vi "Start Condition - Saturation Time (SubVI) (1).vi"(6 "Enum":T1(ring), 8 "error in (no error)":errorcluster, 9 "Time":dbl, 10 "Select":i32, 11 "Cluster in":T2 {"M Event" items=["Stop", "Running", "PID", "Up Limit", "Down Limit", "Load Limit"]; "Test Type" items=["Please Select", "Triaxial Shear", "Triaxial UU", "Shearbox", "Permeability", "Consolidation (Stepped Loading)/Swelling", "Saturation (Incremental)", "User Defined", "UCT", "Isotropic Consolidation", "Swelling Pressure", "B-Check", "Saturation (Step Increment)", "Saturation (Ramp)"]; "Data"."Test Type" items=["Please Select", "Triaxial Shear", "Triaxial UU", "Shearbox", "Permeability", "Consolidation (Stepped Loading)/Swelling", "Saturation (Incremental)", "User Defined", "UCT", "Isotropic Consolidation", "Swelling Pressure", "B-Check", "Saturation (Step Increment)", "Saturation (Ramp)"]}) -> (0 "error out":errorcluster, 3 "Cluster out":T2 {"M Event" items=["Stop", "Running", "PID", "Up Limit", "Down Limit", "Load Limit"]; "Test Type" items=["Please Select", "Triaxial Shear", "Triaxial UU", "Shearbox", "Permeability", "Consolidation (Stepped Loading)/Swelling", "Saturation (Incremental)", "User Defined", "UCT", "Isotropic Consolidation", "Swelling Pressure", "B-Check", "Saturation (Step Increment)", "Saturation (Ramp)"]; "Data"."Test Type" items=["Please Select", "Triaxial Shear", "Triaxial UU", "Shearbox", "Permeability", "Consolidation (Stepped Loading)/Swelling", "Saturation (Incremental)", "User Defined", "UCT", "Isotropic Consolidation", "Swelling Pressure", "B-Check", "Saturation (Step Increment)", "Saturation (Ramp)"]})   [LabVIEW 2019]
uses:
  Controls/RunTest - Data Structure.ctl
  Controls/Test Panel - Data Structure.ctl
  Controls/Station - Test Type.ctl
  <vilib>/Utility/miscctls.llb/LVRowAndColumnTypeDef.ctl
  Controls/RunTest - Calculate Data.ctl
  <vilib>/httpClient/ClientHandle.ctl
  Controls/RunTest - Start Condition.ctl
  Controls/RunTest - Stop Condition.ctl
  Controls/UDP - Event.ctl
  <vilib>/httpClient/LabVIEWHTTPClient.lvlib
types:
  T1 = enum16{"Saturation", "B-Check", "Sat Step", "Sat Ramp"}
  T2 = typedef "RunTest - Data Structure.ctl" = cluster{"Test Plan":string[], "PlanRow":i32, "Device Name":string[], "Timeout":i32, "Start?":bool, "Pause?":bool, "IP Address":string[], "LogRow":i32, "Logtype":u16, "Log Elapse":sgl, "Data":T3, "Stop log?":bool, "tdms":refnum<k34>, "Sensor Data":sgl[], "Start time":timestamp, "Prev Log Elapse":u32, "Plot":u16, "X-Axis":u16[], "Y-Axis":u16[], "XY":cluster{"X":dbl, "Y":dbl}[][], "End Stage?":bool, "1run":bool, "Condition":u16[], "Start Con":bool, "Log Con":bool, "Stop Con":bool, "Start Elapse":dbl, "Start Load":dbl, "Motor":i32, "StartRow":i32, "number log":i32, "Dir":bool, "Start time test":timestamp, "Auto":bool, "Check return?":bool, "Inv":cluster{"M":i32[], "Bool":bool[]}, "tdms temp":refnum<k34>, "Zero?":bool, "Plot Timer":dbl, "1st Run":bool, "TDMS Path":path, "MaxLoad":dbl, "Log Timer":sgl[], "Test Type":T4, "Log Sensor":string[], "Save?":bool, "1st Log":bool, "Y-Axis 2":u16[], "On Y-Axis 2":bool, "Decimal":u8[], "Init":cluster{"PWP TS":sgl, "Load TS":sgl, "Volume TS":sgl, "Disp TS":sgl, "CP":sgl, "Vol In":sgl, "Vol Out":sgl, "Load UCT":sgl, "Disp UCT":sgl, "PWP Sat":sgl, "CP Sat":sgl, "Volume IsoCons":sgl, "PWP IsoCons":sgl, "PWP TUU":sgl, "Load TUU":sgl, "Volume TUU":sgl, "Disp TUU":sgl, "Load Cons":sgl, "Disp Cons":sgl, "Volume Sat":sgl, "Vertical Load SB":sgl, "Vertical Disp SB":sgl, "H Disp SB":sgl, "H Load SB":sgl, "PWP BC":sgl, "CP BC":sgl, "PWP Sat Step":sgl, "CP Sat Step":sgl, "Volume Sat Step":sgl, "PWP Sat Ramp":sgl, "CP Sat Ramp":sgl, "Volume Sat Ramp":sgl}, "Calc":T6, "Device Index":i32[], "Channel Index":i32[], "http ref":T7, "fileid":string, "Step Cons":cluster{"V Stress":sgl, "H Settlement":sgl}, "RunTest":bool, "Graph Last":i32, "Init?":bool, "Datalog":bool[], "Start":T8, "Stop":T9, "Running?":bool, "StartTime":dbl, "Log Prev Time":dbl, "KeyName":string[], "Test RunTime":dbl, "Log Prev Axial":dbl, "M Event":T10[], "Last Log":bool, "popup":bool, "PreStart UU":bool, "PreStart Sat":bool, "PreStart BC":bool, "PreStart Sat Step":bool, "PreStart Sat Ramp":bool, "Prev Sat IP":string}
  T3 = typedef "Test Panel - Data Structure.ctl" = cluster{"Station":string, "Sample ID":string, "Job No":string, "Job Description":string, "Filename":string, "Test Type":T4, "Speciment No":string, "Depth":string, "Height":string, "Diameter/Length":string, "Weight":string, "Test Parameter":string, "Station[]":string[], "Edit Pos":T5, "Edit Pos Prev":T5, "Area":string, "Path":string, "sample_id":string}
  T4 = typedef "Station - Test Type.ctl" = u16
  T5 = typedef "LVRowAndColumnTypeDef.ctl" = cluster{"Row":i32, "Column":i32}
  T6 = typedef "RunTest - Calculate Data.ctl" = cluster{"TS":cluster{"Change PWP":sgl, "Change Vol":sgl, "Axial Load":sgl, "CiL":sgl, "Deviator":sgl, "Axial Strain":sgl, "MaxDeviator":sgl, "SS":sgl, "CAS":sgl}, "TUU":cluster{"Change PWP":sgl, "Axial Load":sgl, "CiL":sgl, "Deviator":sgl, "Axial Strain":sgl, "MaxDeviator":sgl}, "Sat":cluster{"B Value":sgl, "PWP Diss":sgl, "CPP":sgl, "CV":sgl}, "Per":cluster{"Change Vol In":sgl, "Change Vol Out":sgl, "Mean Vol":sgl, "Gradient Pressure":sgl, "Outlet Flow":sgl, "Inlet Flow":sgl, "I X1":sgl, "I X2":sgl, "I Y1":sgl, "I Y2":sgl, "O X1":sgl, "O X2":sgl, "O Y1":sgl, "O Y2":sgl}, "Step Cons":cluster{"V Stress":sgl, "H Settlement":sgl, "Total H Settle":sgl, "Prev Total H":sgl}, "UCT":cluster{"ALC":sgl, "H Change":sgl, "Deviator":sgl, "Axial Strain":sgl, "V Stress":sgl, "MaxDeviator":sgl}, "ISO Cons":cluster{"CPP":sgl, "PWP Diss":sgl, "CV":sgl, "VS":sgl}, "SB":cluster{"Speci LenC":sgl, "Shear Strain":sgl, "H LC":sgl, "Normal Stress":sgl, "Shear Stress":sgl, "MaxShear":sgl}, "BC":cluster{"B Value":sgl, "PWP Diss":sgl, "CPP":sgl, "CV":sgl}, "Sat Step":cluster{"B Value":sgl, "PWP Diss":sgl, "CPP":sgl, "CV":sgl}, "Sat Ramp":cluster{"B Value":sgl, "PWP Diss":sgl, "CPP":sgl, "CV":sgl}, "Prev Log":string[]}
  T7 = typedef "LabVIEWHTTPClient.lvlib/ClientHandle.ctl" = refnum<k1>
  T8 = typedef "RunTest - Start Condition.ctl" = cluster{"Cons":cluster{"VS":dbl, "Delay":bool, "No Delay":dbl}, "Sat":cluster{"CP":dbl, "BP":dbl, "StartBP":bool, "Target CP":bool, "Target BP":bool}, "Iso":cluster{"Select":dbl, "BP":dbl, "IC2":dbl, "IC3":dbl, "IC4":dbl, ". IC6":bool, "IC6":dbl, "IC6-2":dbl, "Time Cond":dbl, "Last PWP":dbl, "Target CP":bool, "Target BP":bool, "NewCP":dbl, "NewBP":dbl, "Noti CP":bool, "Noti BP":bool, "Noti PWP":bool, "PrevSatBP":dbl}, "TS":cluster{"SS":dbl, "Engage":bool, "ES":dbl, "LC":dbl, "PreStart":bool, "Trig SS":bool, "Drain":dbl, "Select":u16, "Max SS .":bool, "MaxSS":dbl}, "TUU":cluster{"SS":dbl, "Engage":bool, "ES":dbl, "LC":dbl, "PreStart":bool, "Trig SS":bool, "CP":dbl, "Delay Value":dbl, "Delay":bool, "CP PID":bool}, "UCT":cluster{"SS":dbl, "Engage":bool, "ES":dbl, "LC":dbl, "PreStart":bool, "Trig SS":bool}, "Enable?":bool, "SB":cluster{"SS":dbl, "Engage":bool, "ES":dbl, "LC":dbl, "PreStart":bool, "Trig SS":bool, "VS":dbl, "Delay Value":dbl, "Delay":bool, "VS PID":bool}, "Perm":cluster{"DP":dbl}, "BC":cluster{"CP":dbl, "Target CP":bool, "Target BP":bool, "CP Inc":dbl, "CP .Init":bool, "CP Init":dbl, "1st BC":bool}, "Sat (Step)":cluster{"Select":dbl, "CP":dbl, "BP":dbl, "EP":dbl, "StartCP":bool, "Target CP":bool, "Target BP":bool}, "Sat (Ramp)":cluster{"Select":dbl, "CP":dbl, "BP":dbl, "EP":dbl, "StartCP":bool, "Target CP":bool, "Target BP":bool, "Time Rate":u32}}
  T9 = typedef "RunTest - Stop Condition.ctl" = cluster{"Cons":cluster{"Select":i32, "Disp":dbl, "Time":dbl, "Time2":dbl, "Disp 2":dbl, "Time Cond":dbl, "Last Disp":dbl, "Swell":bool, "T50,90,100":cluster{"t50_x_min":dbl, "t50_y_value":dbl, "t90_x_min":dbl, "t90_y_value":dbl, "t100_x_min":dbl, "t100_y_value":dbl, "target_column":string, "test_type":string, "error":string}}, "Sat":cluster{"Select":i32, "PP":dbl, "Time":dbl, "VC":dbl, "Time2":dbl, "Time Cond":dbl, "Last PP":dbl, ".B":bool, "B":dbl, "Last Vc":dbl, "Time Cond 2":dbl, "Time3":dbl, "Time Cond 3":dbl, "B Achieve":bool, "PP Achieve":bool, "VC Achieve":bool, "Max Achieve":bool, "CP Check":dbl, "Skip Next":bool, "B Achieve Stage":u32, ".CP Check":bool}, "Iso":cluster{"PP":dbl, "Time":dbl, "VC":dbl, "Time2":dbl, "Time Cond":dbl, "Last Vc":dbl, ".PP":bool, "Time Cond 2":dbl, "Select":i32, "BS":cluster{"t50_x_min":dbl, "t50_y_value":dbl, "t90_x_min":dbl, "t90_y_value":dbl, "t100_x_min":dbl, "t100_y_value":dbl, "target_column":string, "test_type":string, "error":string}, "Final VC":dbl, "ASTM":cluster{"t50_x_min":dbl, "t50_y_value":dbl, "t90_x_min":dbl, "t90_y_value":dbl, "t100_x_min":dbl, "t100_y_value":dbl, "target_column":string, "test_type":string, "error":string}, "ASTM Log":cluster{"t50_x_min":dbl, "t50_y_value":dbl, "t90_x_min":dbl, "t90_y_value":dbl, "t100_x_min":dbl, "t100_y_value":dbl, "target_column":string, "test_type":string, "error":string}, "PP Achieve":bool, "VC Achieve":bool}, "TS":cluster{"Axial":dbl, ".MaxDev":bool, "MaxDev Value":dbl, "Return":bool, "Reset":bool, "Prev Time":dbl, "PostStop Run":bool, "CP Stop":bool, "BP Stop":bool, "PostStop Trig":bool, "Reset Value":dbl, "BPTrig":bool, "CPTrig":bool, "VLCTrig":bool, "CAxial":dbl, "Select":i32}, "TUU":cluster{"Axial":dbl, ".MaxDev":bool, "MaxDev Value":dbl, "Return":bool, "Reset":bool, "Prev Time":dbl, "PostStop Run":bool, "CP Stop":bool, "BP Stop":bool, "PostStop Trig":bool, "Reset Value":dbl, "BPTrig":bool, "CPTrig":bool, "VLCTrig":bool}, "UCT":cluster{"Axial":dbl, ".MaxDev":bool, "MaxDev Value":dbl, "Return":bool, "Reset":bool, "Prev Time":dbl, "PostStop Run":bool, "CP Stop":bool, "BP Stop":bool, "PostStop Trig":bool}, "Enable?":bool, "SB":cluster{"Shear":dbl, ".MaxShear":bool, "MaxShear Value":dbl, "Return":bool, "Reset":bool, "Prev Time":dbl, "PostStop Run":bool, "CP Stop":bool, "BP Stop":bool, "PostStop Trig":bool, "Reset Value":dbl, "BPTrig":bool, "CPTrig":bool, "VLCTrig":bool}, "Perm":cluster{"Max Time":bool, "Reset":bool, "PostStop Run":bool, "Ratio":bool, "Reset Value":dbl, "Time":dbl, "RatioTime":dbl, "RatioMore":dbl, "RatioLess":dbl, "Time Cond":dbl, "Time Cond 2":dbl, "Prev IF":dbl, "Prev OF":dbl, "PostStop Trig":bool, "BP Trig":bool, "DP Stop":bool, "BP Stop":bool, "CP Stop":bool, "CP Trig":bool}, "SP":cluster{".Max Time":bool, ".Time":bool, "Time":dbl, "MaxTime":dbl, "Time Cond":dbl, "Max Time Cond":dbl, "Stress":dbl}, "BC":cluster{"Select":i32, "PP":dbl, "Time":dbl, "Time Cond":dbl, "Last PP":dbl, ".B":bool, "B":dbl, "Time 2":dbl, "Time Cond 2":dbl, "B Achieve":bool, "PP Achieve":bool, "Max Achieve":bool, "CP Check":dbl, "Skip Next":bool, "B Achieve Stage":u32, ".CP Check":bool}, "Sat (Step)":cluster{"Select":i32, "PP":dbl, "Time":dbl, "VC":dbl, "Time2":dbl, "Time Cond":dbl, "Last PP":dbl, ".B":bool, "B":dbl, "Last Vc":dbl, "Time Cond 2":dbl, "Time3":dbl, "Time Cond 3":dbl, "B Achieve":bool, "PP Achieve":bool, "VC Achieve":bool, "Max Achieve":bool, "CP Check":dbl, "Skip Next":bool, "B Achieve Stage":u32}, "Sat (Ramp)":cluster{"Select":i32, "PP":dbl, "Time":dbl, "VC":dbl, "Time2":dbl, "Time Cond":dbl, "Last PP":dbl, ".B":bool, "B":dbl, "Last Vc":dbl, "Time Cond 2":dbl, "Time3":dbl, "Time Cond 3":dbl, "B Achieve":bool, "PP Achieve":bool, "VC Achieve":bool, "Max Achieve":bool, "CP Check":dbl, "Skip Next":bool, "B Achieve Stage":u32}}
  T10 = typedef "UDP - Event.ctl" = u16
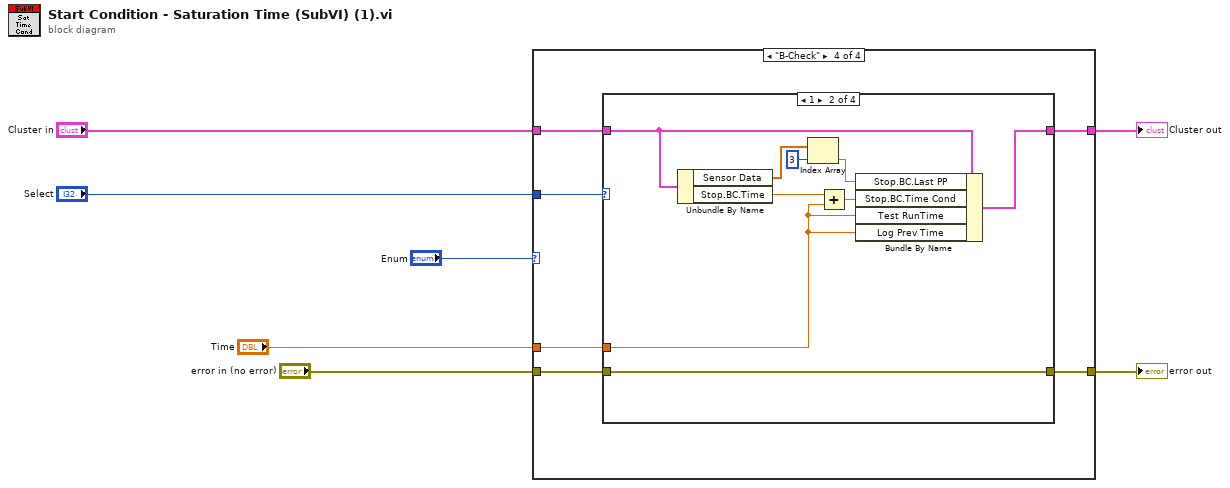
[diagram p0: block diagram]
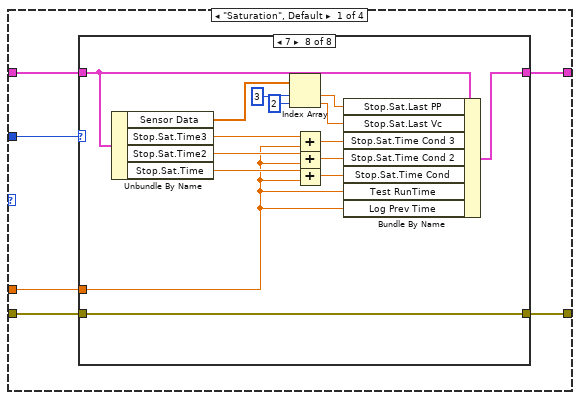
[diagram p2: hidden frame]
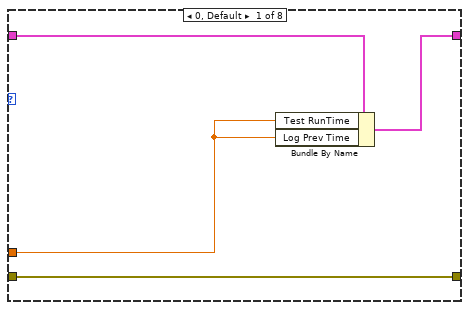
[diagram p3: hidden frame]
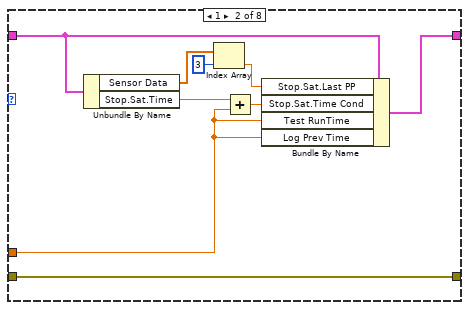
[diagram p4: hidden frame]
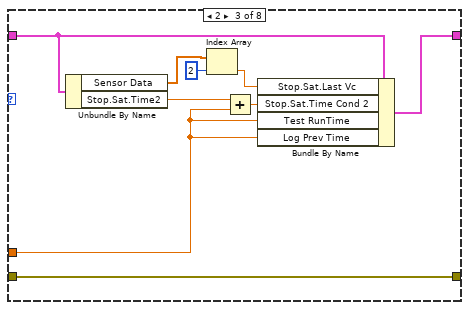
[diagram p5: hidden frame]
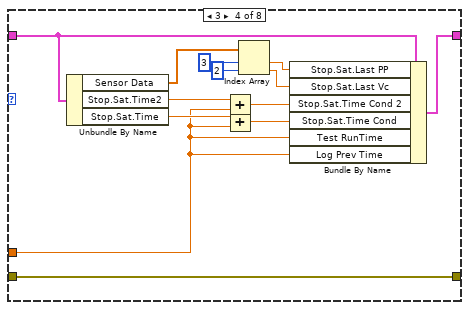
[diagram p6: hidden frame]
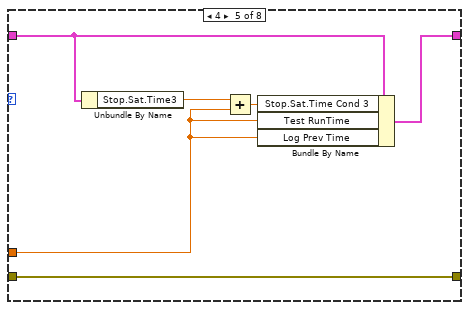
[diagram p7: hidden frame]
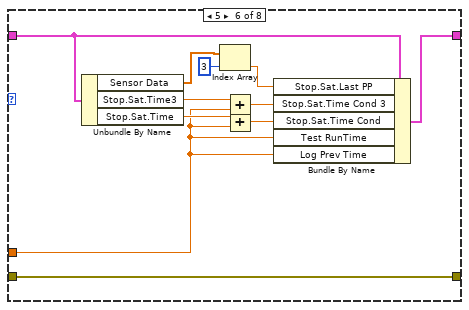
[diagram p8: hidden frame]
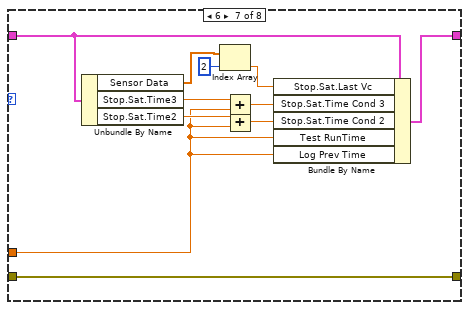
[diagram p9: hidden frame]
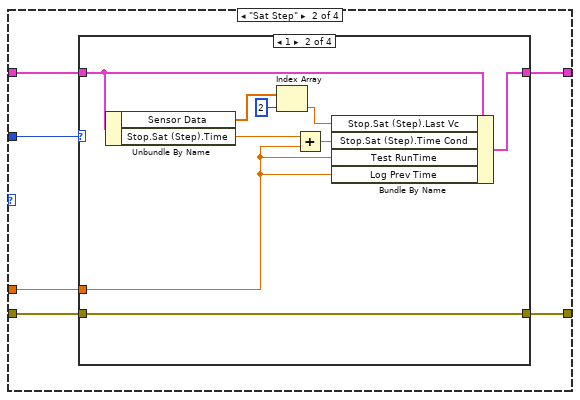
[diagram p10: hidden frame]
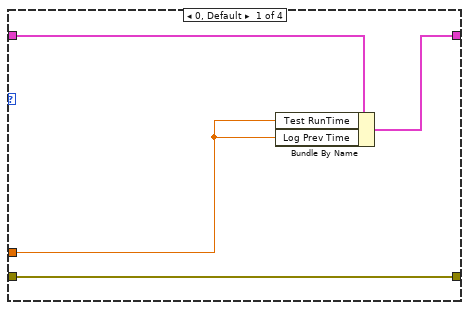
[diagram p11: hidden frame]
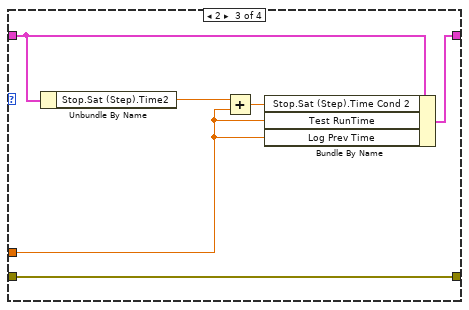
[diagram p12: hidden frame]
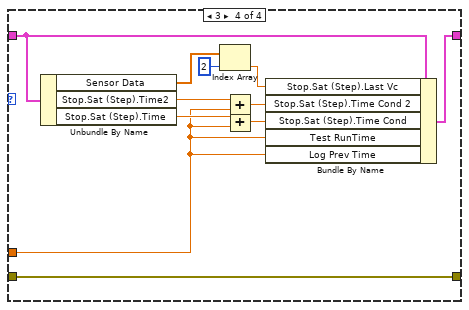
[diagram p13: hidden frame]
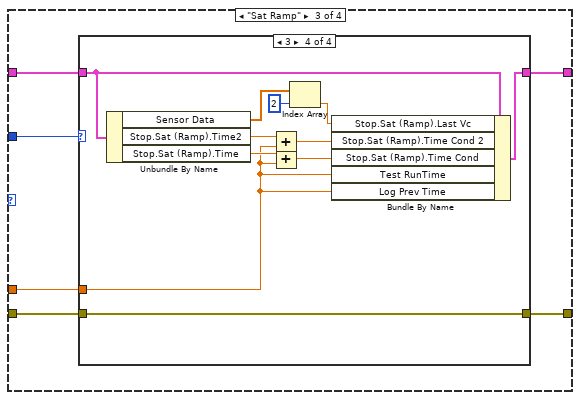
[diagram p14: hidden frame]
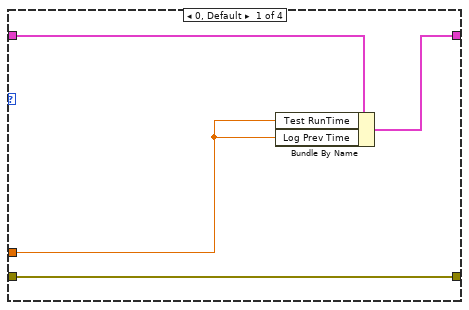
[diagram p15: hidden frame]
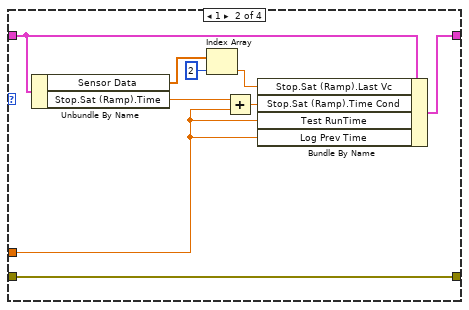
[diagram p16: hidden frame]
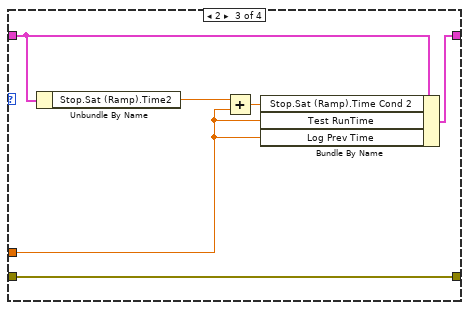
[diagram p17: hidden frame]
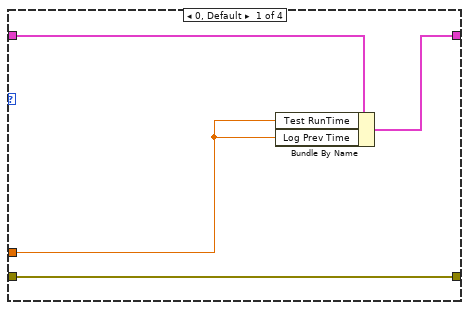
[diagram p18: hidden frame]
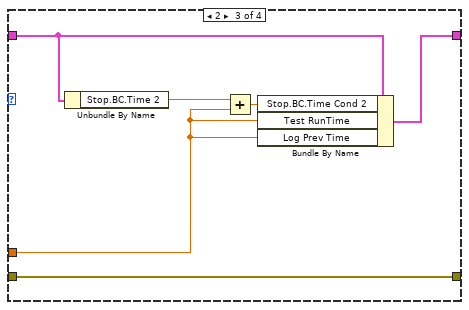
[diagram p19: hidden frame]
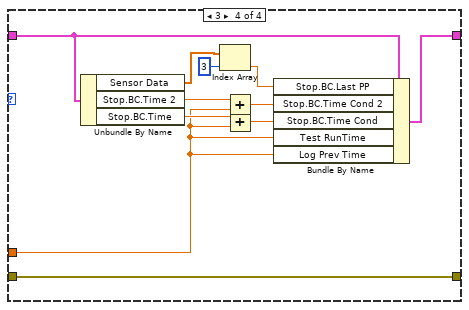
[diagram p20: hidden frame]
diagram:
  n1 = case shown="\"B-Check\"" "Enum" {
    tunnel: "error in (no error)" -> [w13 w97 w133 w169]
    tunnel: [w12 w96 w132 w168] -> w6
    tunnel: "Time" -> [w11 w95 w131 w167]
    tunnel: "Cluster in" -> [w10 w94 w130 w166]
    tunnel: "Select" -> [w9 w93 w129 w165]
    tunnel: [w8 w92 w128 w164] -> w2
    frame "Saturation", Default {
      n2 = case shown="7" w9 {
        tunnel: w11 -> [w15 w22 w31 w36 w50 w55 w66 w78]
        tunnel: [w17 w26 w35 w48 w54 w65 w76 w91] -> w8
        tunnel: w10 -> [w16 w24 w33 w46 w52 w63 w74 w90]
        tunnel: [w14 w18 w27 w41 w49 w61 w72 w88] -> w12
        tunnel: w13 -> [w14 w18 w27 w41 w49 w61 w72 w88]
        frame 0, Default {
          n3 = Bundle By Name(cluster=w16, "Test RunTime"=w15, "Log Prev Time"=w15) -> (w17:T2)
        }
        frame 1 {
          n4 = Unbundle By Name(w24) -> ("Sensor Data"=w20:sgl[], "Stop.Sat.Time"=w23:dbl)
          n5 = Index Array(array=w20, index=3) -> (element=w19:sgl)
          n6 = Add(x=w23, y=w22) -> (x+y=w25:dbl)
          n7 = Bundle By Name(cluster=w24, "Stop.Sat.Last PP"=w19, "Stop.Sat.Time Cond"=w25, "Test RunTime"=w22, "Log Prev Time"=w22) -> (w26:T2)
        }
        frame 2 {
          n8 = Unbundle By Name(w33) -> ("Sensor Data"=w29:sgl[], "Stop.Sat.Time2"=w32:dbl)
          n9 = Index Array(array=w29, index=2) -> (element=w28:sgl)
          n10 = Add(x=w32, y=w31) -> (x+y=w34:dbl)
          n11 = Bundle By Name(cluster=w33, "Stop.Sat.Last Vc"=w28, "Stop.Sat.Time Cond 2"=w34, "Test RunTime"=w31, "Log Prev Time"=w31) -> (w35:T2)
        }
        frame 3 {
          n12 = Unbundle By Name(w46) -> ("Sensor Data"=w43:sgl[], "Stop.Sat.Time2"=w45:dbl, "Stop.Sat.Time"=w37:dbl)
          n13 = Add(x=w45, y=w36) -> (x+y=w47:dbl)
          n14 = Add(x=w37, y=w36) -> (x+y=w38:dbl)
          n15 = Index Array(array=w43, index #1=3 ("index"), index #2=2 ("index")) -> (element #1=w39:sgl, element #2=w42:sgl)
          n16 = Bundle By Name(cluster=w46, "Stop.Sat.Last PP"=w39, "Stop.Sat.Last Vc"=w42, "Stop.Sat.Time Cond 2"=w47, "Stop.Sat.Time Cond"=w38, "Test RunTime"=w36, "Log Prev Time"=w36) -> (w48:T2)
        }
        frame 4 {
          n17 = Unbundle By Name(w52) -> ("Stop.Sat.Time3"=w51:dbl)
          n18 = Add(x=w51, y=w50) -> (x+y=w53:dbl)
          n19 = Bundle By Name(cluster=w52, "Stop.Sat.Time Cond 3"=w53, "Test RunTime"=w50, "Log Prev Time"=w50) -> (w54:T2)
        }
        frame 5 {
          n20 = Unbundle By Name(w63) -> ("Sensor Data"=w59:sgl[], "Stop.Sat.Time3"=w62:dbl, "Stop.Sat.Time"=w56:dbl)
          n21 = Index Array(array=w59, index=3) -> (element=w58:sgl)
          n22 = Add(x=w62, y=w55) -> (x+y=w64:dbl)
          n23 = Add(x=w56, y=w55) -> (x+y=w57:dbl)
          n24 = Bundle By Name(cluster=w63, "Stop.Sat.Last PP"=w58, "Stop.Sat.Time Cond 3"=w64, "Stop.Sat.Time Cond"=w57, "Test RunTime"=w55, "Log Prev Time"=w55) -> (w65:T2)
        }
        frame 6 {
          n25 = Unbundle By Name(w74) -> ("Sensor Data"=w70:sgl[], "Stop.Sat.Time3"=w73:dbl, "Stop.Sat.Time2"=w67:dbl)
          n26 = Index Array(array=w70, index=2) -> (element=w69:sgl)
          n27 = Add(x=w73, y=w66) -> (x+y=w75:dbl)
          n28 = Add(x=w67, y=w66) -> (x+y=w68:dbl)
          n29 = Bundle By Name(cluster=w74, "Stop.Sat.Last Vc"=w69, "Stop.Sat.Time Cond 3"=w75, "Stop.Sat.Time Cond 2"=w68, "Test RunTime"=w66, "Log Prev Time"=w66) -> (w76:T2)
        }
        frame 7 {
          n30 = Unbundle By Name(w90) -> ("Sensor Data"=w86:sgl[], "Stop.Sat.Time3"=w89:dbl, "Stop.Sat.Time2"=w81:dbl, "Stop.Sat.Time"=w79:dbl)
          n31 = Index Array(array=w86, index #1=3 ("index"), index #2=2 ("index")) -> (element #1=w82:sgl, element #2=w85:sgl)
          n32 = Add(x=w89, y=w78) -> (x+y=w80:dbl)
          n33 = Add(x=w81, y=w78) -> (x+y=w84:dbl)
          n34 = Add(x=w79, y=w78) -> (x+y=w77:dbl)
          n35 = Bundle By Name(cluster=w90, "Stop.Sat.Last PP"=w82, "Stop.Sat.Last Vc"=w85, "Stop.Sat.Time Cond 3"=w80, "Stop.Sat.Time Cond 2"=w84, "Stop.Sat.Time Cond"=w77, "Test RunTime"=w78, "Log Prev Time"=w78) -> (w91:T2)
        }
      }
    }
    frame "Sat Step" {
      n36 = case shown="1" w93 {
        tunnel: w95 -> [w99 w106 w112 w117]
        tunnel: [w101 w110 w116 w127] -> w92
        tunnel: w94 -> [w100 w108 w114 w125]
        tunnel: [w98 w102 w111 w123] -> w96
        tunnel: w97 -> [w98 w102 w111 w123]
        frame 0, Default {
          n37 = Bundle By Name(cluster=w100, "Test RunTime"=w99, "Log Prev Time"=w99) -> (w101:T2)
        }
        frame 1 {
          n38 = Unbundle By Name(w108) -> ("Sensor Data"=w104:sgl[], "Stop.Sat (Step).Time"=w107:dbl)
          n39 = Index Array(array=w104, index=2) -> (element=w103:sgl)
          n40 = Add(x=w107, y=w106) -> (x+y=w109:dbl)
          n41 = Bundle By Name(cluster=w108, "Stop.Sat (Step).Last Vc"=w103, "Stop.Sat (Step).Time Cond"=w109, "Test RunTime"=w106, "Log Prev Time"=w106) -> (w110:T2)
        }
        frame 2 {
          n42 = Unbundle By Name(w114) -> ("Stop.Sat (Step).Time2"=w113:dbl)
          n43 = Add(x=w113, y=w112) -> (x+y=w115:dbl)
          n44 = Bundle By Name(cluster=w114, "Stop.Sat (Step).Time Cond 2"=w115, "Test RunTime"=w112, "Log Prev Time"=w112) -> (w116:T2)
        }
        frame 3 {
          n45 = Unbundle By Name(w125) -> ("Sensor Data"=w121:sgl[], "Stop.Sat (Step).Time2"=w124:dbl, "Stop.Sat (Step).Time"=w118:dbl)
          n46 = Index Array(array=w121, index=2) -> (element=w120:sgl)
          n47 = Add(x=w124, y=w117) -> (x+y=w126:dbl)
          n48 = Add(x=w118, y=w117) -> (x+y=w119:dbl)
          n49 = Bundle By Name(cluster=w125, "Stop.Sat (Step).Last Vc"=w120, "Stop.Sat (Step).Time Cond 2"=w126, "Stop.Sat (Step).Time Cond"=w119, "Test RunTime"=w117, "Log Prev Time"=w117) -> (w127:T2)
        }
      }
    }
    frame "Sat Ramp" {
      n50 = case shown="3" w129 {
        tunnel: w131 -> [w135 w142 w148 w153]
        tunnel: [w137 w146 w152 w163] -> w128
        tunnel: w130 -> [w136 w144 w150 w161]
        tunnel: [w134 w138 w147 w159] -> w132
        tunnel: w133 -> [w134 w138 w147 w159]
        frame 0, Default {
          n51 = Bundle By Name(cluster=w136, "Test RunTime"=w135, "Log Prev Time"=w135) -> (w137:T2)
        }
        frame 1 {
          n52 = Unbundle By Name(w144) -> ("Sensor Data"=w140:sgl[], "Stop.Sat (Ramp).Time"=w143:dbl)
          n53 = Index Array(array=w140, index=2) -> (element=w139:sgl)
          n54 = Add(x=w143, y=w142) -> (x+y=w145:dbl)
          n55 = Bundle By Name(cluster=w144, "Stop.Sat (Ramp).Last Vc"=w139, "Stop.Sat (Ramp).Time Cond"=w145, "Test RunTime"=w142, "Log Prev Time"=w142) -> (w146:T2)
        }
        frame 2 {
          n56 = Unbundle By Name(w150) -> ("Stop.Sat (Ramp).Time2"=w149:dbl)
          n57 = Add(x=w149, y=w148) -> (x+y=w151:dbl)
          n58 = Bundle By Name(cluster=w150, "Stop.Sat (Ramp).Time Cond 2"=w151, "Test RunTime"=w148, "Log Prev Time"=w148) -> (w152:T2)
        }
        frame 3 {
          n59 = Unbundle By Name(w161) -> ("Sensor Data"=w157:sgl[], "Stop.Sat (Ramp).Time2"=w160:dbl, "Stop.Sat (Ramp).Time"=w154:dbl)
          n60 = Add(x=w160, y=w153) -> (x+y=w162:dbl)
          n61 = Add(x=w154, y=w153) -> (x+y=w155:dbl)
          n62 = Index Array(array=w157, index=2) -> (element=w156:sgl)
          n63 = Bundle By Name(cluster=w161, "Stop.Sat (Ramp).Last Vc"=w156, "Stop.Sat (Ramp).Time Cond 2"=w162, "Stop.Sat (Ramp).Time Cond"=w155, "Test RunTime"=w153, "Log Prev Time"=w153) -> (w163:T2)
        }
      }
    }
    frame "B-Check" {
      n64 = case shown="1" w165 {
        tunnel: w167 -> [w171 w178 w184 w189]
        tunnel: [w173 w182 w188 w199] -> w164
        tunnel: w166 -> [w172 w180 w186 w197]
        tunnel: [w170 w174 w183 w195] -> w168
        tunnel: w169 -> [w170 w174 w183 w195]
        frame 0, Default {
          n65 = Bundle By Name(cluster=w172, "Test RunTime"=w171, "Log Prev Time"=w171) -> (w173:T2)
        }
        frame 1 {
          n66 = Unbundle By Name(w180) -> ("Sensor Data"=w176:sgl[], "Stop.BC.Time"=w179:dbl)
          n67 = Index Array(array=w176, index=3) -> (element=w175:sgl)
          n68 = Add(x=w179, y=w178) -> (x+y=w181:dbl)
          n69 = Bundle By Name(cluster=w180, "Stop.BC.Last PP"=w175, "Stop.BC.Time Cond"=w181, "Test RunTime"=w178, "Log Prev Time"=w178) -> (w182:T2)
        }
        frame 2 {
          n70 = Unbundle By Name(w186) -> ("Stop.BC.Time 2"=w185:dbl)
          n71 = Add(x=w185, y=w184) -> (x+y=w187:dbl)
          n72 = Bundle By Name(cluster=w186, "Stop.BC.Time Cond 2"=w187, "Test RunTime"=w184, "Log Prev Time"=w184) -> (w188:T2)
        }
        frame 3 {
          n73 = Unbundle By Name(w197) -> ("Sensor Data"=w193:sgl[], "Stop.BC.Time 2"=w196:dbl, "Stop.BC.Time"=w190:dbl)
          n74 = Index Array(array=w193, index=3) -> (element=w192:sgl)
          n75 = Add(x=w196, y=w189) -> (x+y=w198:dbl)
          n76 = Add(x=w190, y=w189) -> (x+y=w191:dbl)
          n77 = Bundle By Name(cluster=w197, "Stop.BC.Last PP"=w192, "Stop.BC.Time Cond 2"=w198, "Stop.BC.Time Cond"=w191, "Test RunTime"=w189, "Log Prev Time"=w189) -> (w199:T2)
        }
      }
    }
  }
  "error out" <- w6
  "Cluster out" <- w2
